vi "FuncVI-MsgBox.vi"(5 "InstanceRef":T2, 9 "arg list":T1[](array[typedef]) {"num" format="%.2f"}) -> (0 "error out":bool, 3 "result":T1 {"num" format="%.2f"})   [LabVIEW 2021]
doc: "::: CalcExpress Toolkit :::\nCopyright (c) 2000-2026 Konstantin Shifershteyn. All rights reserved."
uses:
  cetypes.llb/CalcExpress Function Argument Info.ctl
  cetypes.llb/CalcExpress Instance RefNum.ctl
panel:
  in  "max arg num":i32=1000
  in  "min arg num":i32
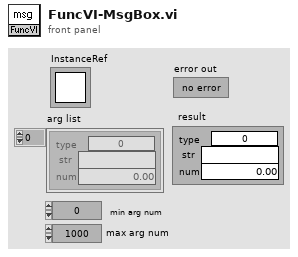
[diagram p1: front panel]
types:
  T1 = typedef "CalcExpress Function Argument Info.ctl" = cluster{"type":u32, "str":string, "num":dbl}
  T2 = typedef "CalcExpress Instance RefNum.ctl" = refnum<k1>
  T3 = enum8{"String", "DBL Number", "identifier", "1D Array of DBL", "2D Array of DBL", "CDB Number", "1D Array of CDB", "2D Array of CDB", "1D Array of String", "2D Array of String", "Unknown data type"}
  T4 = cluster{"type":enum8{"String", "DBL Number", "identifier", "1D Array of DBL", "2D Array of DBL", "CDB Number", "1D Array of CDB", "2D Array of CDB", "1D Array of String", "2D Array of String", "Unknown data type"}, string, "return value":dbl}
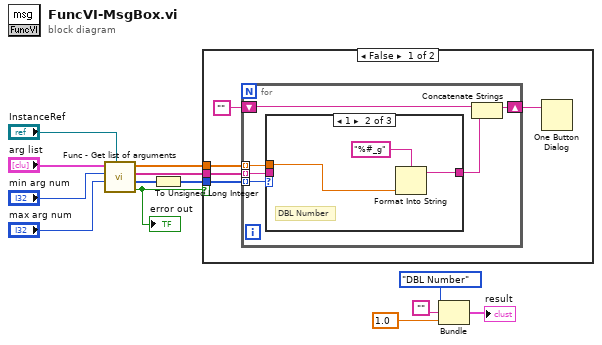
[diagram p0: block diagram]
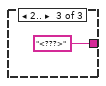
[diagram p3: hidden frame]
diagram:
  n1 = call "Func - Get list of arguments.vi"("InstanceRef"="InstanceRef", "max arg num"="max arg num", "min arg num"="min arg num", "arg list"="arg list") -> ("error out"=w8:bool, "type list"=w11:u32[], "str list"=w12:string[], "num list"=w13:dbl[])  [unwired: 4 in]
  "error out" <- w8
  n2 = To Unsigned Long Integer(number=w11) -> (unsigned 32bit integer=w4:u32[])
  n3 = case shown="False" w8 {
    tunnel: w4 -> [w18 _]
    tunnel: w12 -> [w17 _]
    tunnel: w13 -> [w16 _]
    frame False {
      n4 = for {
        tunnel: w16 -> [w24] mode=indexing
        tunnel: w17 -> [w23] mode=indexing
        tunnel: w18 -> [w22] mode=indexing
        shift-right: [w20] -> w14
        shift-left: "" -> [w21]
        n5 = case shown="1" w22 {
          tunnel: [w25 w27 "<???>" ("str")] -> w19
          tunnel: w23 -> [w25 _ _]
          tunnel: w24 -> [_ w26 _]
          frame ..0 {
            # "String"
          }
          frame 1 {
            # "DBL Number"
            n6 = Format Into String(format string="%#_g", w26) -> (resulting string=w27:string)  [unwired: 2 in, 1 out]
          }
          frame 2.. {
          }
        }
        n7 = Concatenate Strings(w21, w19) -> (w20:string)
      }
      n8 = One Button Dialog(message=w14) -> ()  [unwired: 1 in, 1 out]
    }
    frame True {
    }
  }
  n9 = Bundle("type"=T3."DBL Number", "", "return value"=1.0) -> (→"result":T4)  [unwired: 1 in]
